vi "PIDController_AdvCalculate_FF_Sp_Pv_Per.vi"(6 "Period":dbl, 7 "Auto":bool=TRUE, 8 "FF":dbl, 9 "SP":dbl, 10 "PV":dbl, 11 "in PID_CONTROLLER":T1={"Kp"=0.0, "Ki"=0.0, "Kd"=0.0, "Period"=0.0, "Max_Integral"=0.0, "Min_Integral"=0.0, "Max_Input"=0.0, "Min_Input"=0.0, "Continuous"=FALSE, "PositionError"=0.0, "VelocityError"=0.0, "PrevError"=0.0, "Total_Integral"=0.0, "PositionTolerance"=0.0, "VelocityTolerance"=0.0, "SetPoint"=0.0, "Kf"=0.0, "Prev_Deriv"=0.0, "Prev_Deriv 2"=0.0, "DerivativeFilter"=FALSE, "Min_Output"=-9.99e+35, "Max_Output"=9.9e+35, "Prev_F_P"=0.0, "Prev_F_P_2"=0.0, "AntiWindupActive"=FALSE, "Measurement"=0.0, "IntegralZone"=9.9e+30} {"IntegralZone" format="%16_6e"; "Measurement" format="%16_6e"; "Prev_F_P_2" format="%16_6e"; "Prev_F_P" format="%16_6e"; "Max_Output" format="%16_6e"; "Min_Output" format="%16_6e"; "Prev_Deriv 2" format="%16_6e"; "Prev_Deriv" format="%16_6e"; "Kf" format="%16_6e"; "SetPoint" format="%16_6e"; "VelocityTolerance" format="%16_6e"; "PositionTolerance" format="%16_6e"; "Total_Integral" format="%16_6e"; "PrevError" format="%16_6e"; "VelocityError" format="%16_6e"; "PositionError" format="%16_6e"; "Min_Input" format="%16_6e"; "Max_Input" format="%16_6e"; "Min_Integral" format="%16_6e"; "Max_Integral" format="%16_6e"; "Period" format="%16_6e"; "Kd" format="%16_6e"; "Ki" format="%16_6e"; "Kp" format="%16_6e"}) -> (1 "ControlOutput":dbl, 3 "out PID_CONTROLLER":T1={"Kp"=0.0, "Ki"=0.0, "Kd"=0.0, "Period"=0.0, "Max_Integral"=0.0, "Min_Integral"=0.0, "Max_Input"=0.0, "Min_Input"=0.0, "Continuous"=FALSE, "PositionError"=0.0, "VelocityError"=0.0, "PrevError"=0.0, "Total_Integral"=0.0, "PositionTolerance"=0.0, "VelocityTolerance"=0.0, "SetPoint"=0.0, "Kf"=0.0, "Prev_Deriv"=0.0, "Prev_Deriv 2"=0.0, "DerivativeFilter"=FALSE, "Min_Output"=-9.99e+35, "Max_Output"=9.9e+35, "Prev_F_P"=0.0, "Prev_F_P_2"=0.0, "AntiWindupActive"=FALSE, "Measurement"=0.0, "IntegralZone"=9.9e+30} {"IntegralZone" format="%16_6e"; "Measurement" format="%16_6e"; "Prev_F_P_2" format="%16_6e"; "Prev_F_P" format="%16_6e"; "Max_Output" format="%16_6e"; "Min_Output" format="%16_6e"; "Prev_Deriv 2" format="%16_6e"; "Prev_Deriv" format="%16_6e"; "Kf" format="%16_6e"; "SetPoint" format="%16_6e"; "VelocityTolerance" format="%16_6e"; "PositionTolerance" format="%16_6e"; "Total_Integral" format="%16_6e"; "PrevError" format="%16_6e"; "VelocityError" format="%16_6e"; "PositionError" format="%16_6e"; "Min_Input" format="%16_6e"; "Max_Input" format="%16_6e"; "Min_Integral" format="%16_6e"; "Max_Integral" format="%16_6e"; "Period" format="%16_6e"; "Kd" format="%16_6e"; "Ki" format="%16_6e"; "Kp" format="%16_6e"})   [LabVIEW 2019, in "Trajectory_Library.lvlib"]
doc: "Returns the next output of the \"advanced\" PID controller. This controller implements the same PID as the \"normal\" controller with the following enhancements:\n - Integration by trapezoids is used.\n - Optionally filters derivative terms. (See SetDerivativeFilter subVI documentation for information.)\n - Incorporates optional feedforward.\n - Includes integral windup protection. This is only useful when output limits are specified.\n - When not called with a specific period, uses the actual elapsed time. (This subVI requires the call to pass the time period.) \n - Limits the outputs. When output limits are specified the output is cooerced be within these limits.\n - Includes an Auto/Manual mode. In manual mode the scaled feedforward is sent directly to the output and the PID controller tracks this output value to allow for smooth transition back to auto mode.\n\nThe generalized equation for this PID when in auto is:\n CO = Kf x feedforward + Kp x error + Ki x Integral(error) + Kd x Derivative(error)\n\nWhen auto mode is disabled, the generaized equation is:\n CO = Kf x feedforward \n \nInputs:\n - PID_Controller -- PID_Controller data cluster\n - PV-measurement -- The current measurement of the process variable. (PV)\n - SP-setpoint -- The new setpoint of the controller. (SP)\n - FF-feedforward -- Feedforward n the same units as the PV and SP\n - Period -- Period of this controller in seconds.\n - Auto -- Use the PID calculate when this is True\n\nOutputs:\n - PID_Controller -- Updated PID_Controller data cluster\n - CO-ControlOutput -- Controller output (CO)"
uses:
  Trajectory_Library.lvlib
  TypeDef/PID_CONTROLLER.ctl
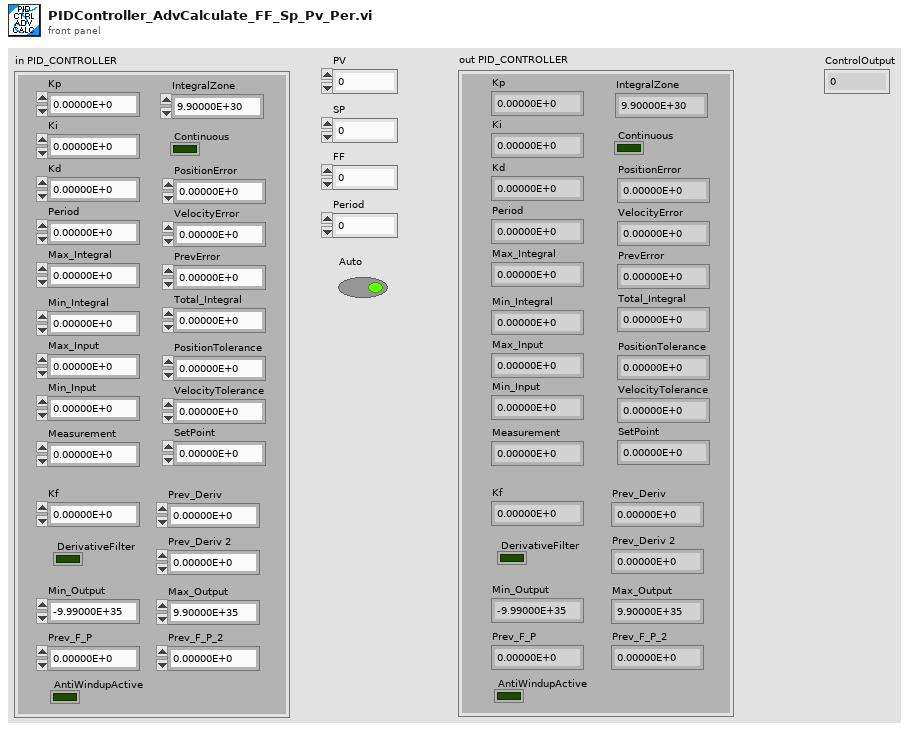
[diagram p1: front panel]
types:
  T1 = typedef "Trajectory_Library.lvlib/PID_CONTROLLER.ctl" = cluster{"Kp":dbl, "Ki":dbl, "Kd":dbl, "Period":dbl, "Max_Integral":dbl, "Min_Integral":dbl, "Max_Input":dbl, "Min_Input":dbl, "Continuous":bool, "PositionError":dbl, "VelocityError":dbl, "PrevError":dbl, "Total_Integral":dbl, "PositionTolerance":dbl, "VelocityTolerance":dbl, "SetPoint":dbl, "Kf":dbl, "Prev_Deriv":dbl, "Prev_Deriv 2":dbl, "DerivativeFilter":bool, "Min_Output":dbl, "Max_Output":dbl, "Prev_F_P":dbl, "Prev_F_P_2":dbl, "AntiWindupActive":bool, "Measurement":dbl, "IntegralZone":dbl}
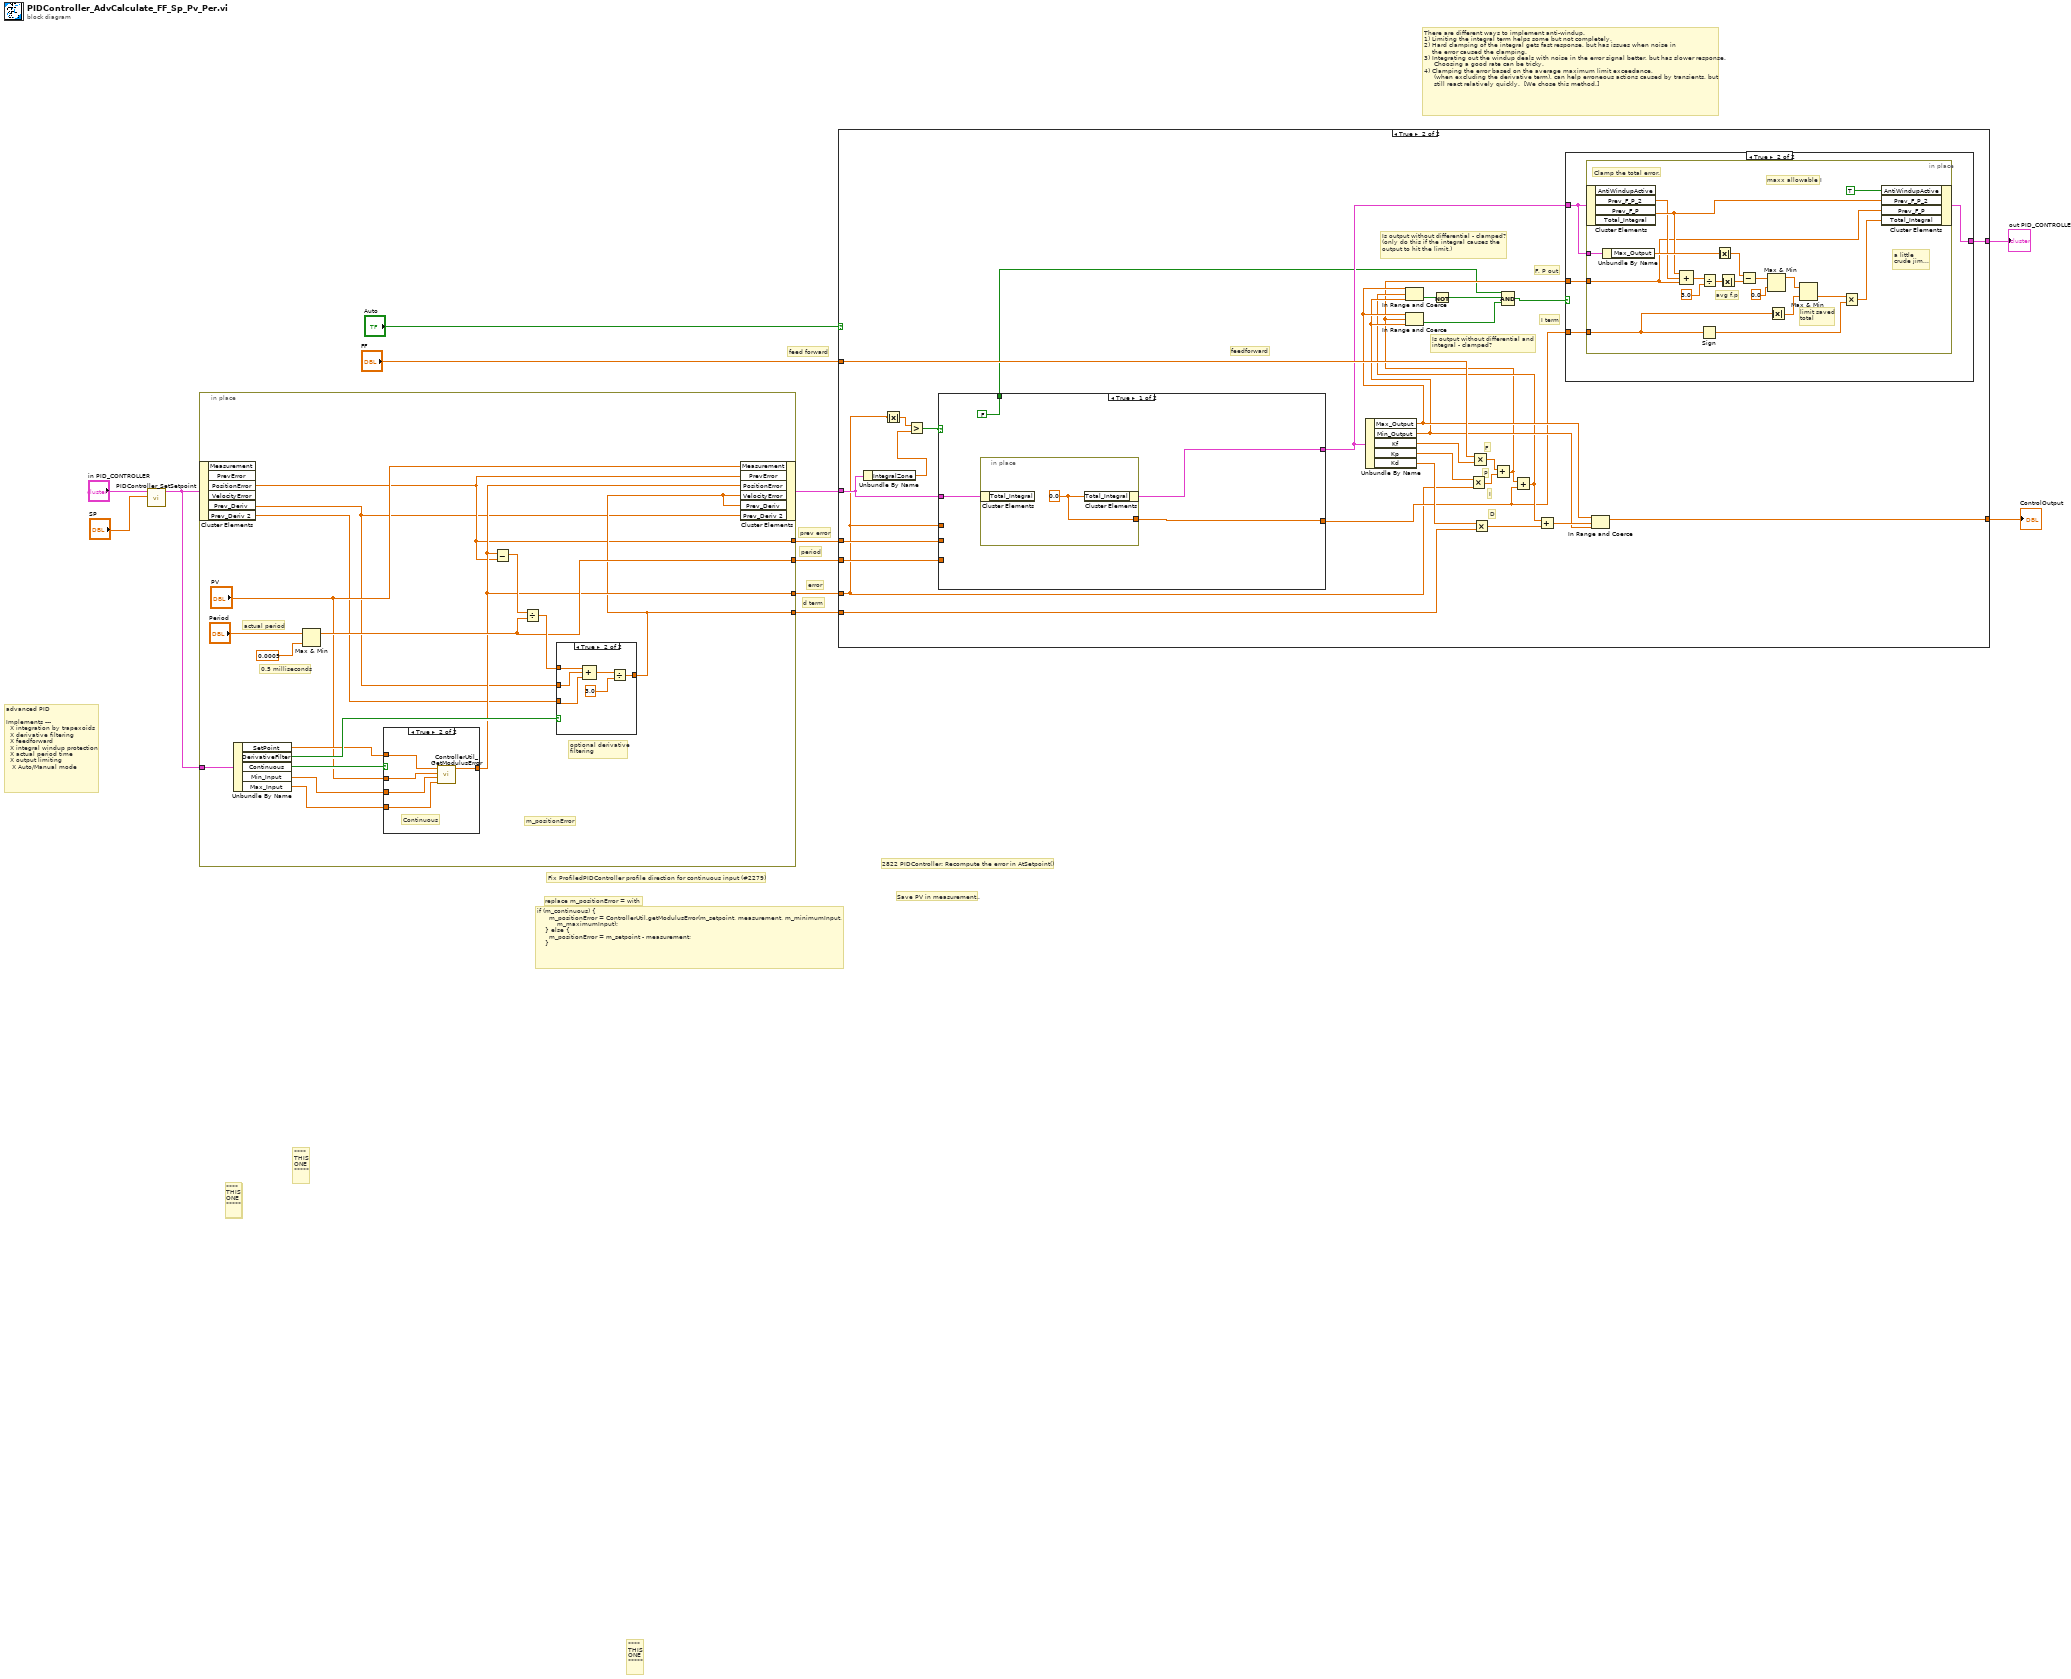
[diagram p0: block diagram]
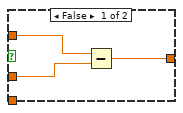
[diagram p2: hidden frame]
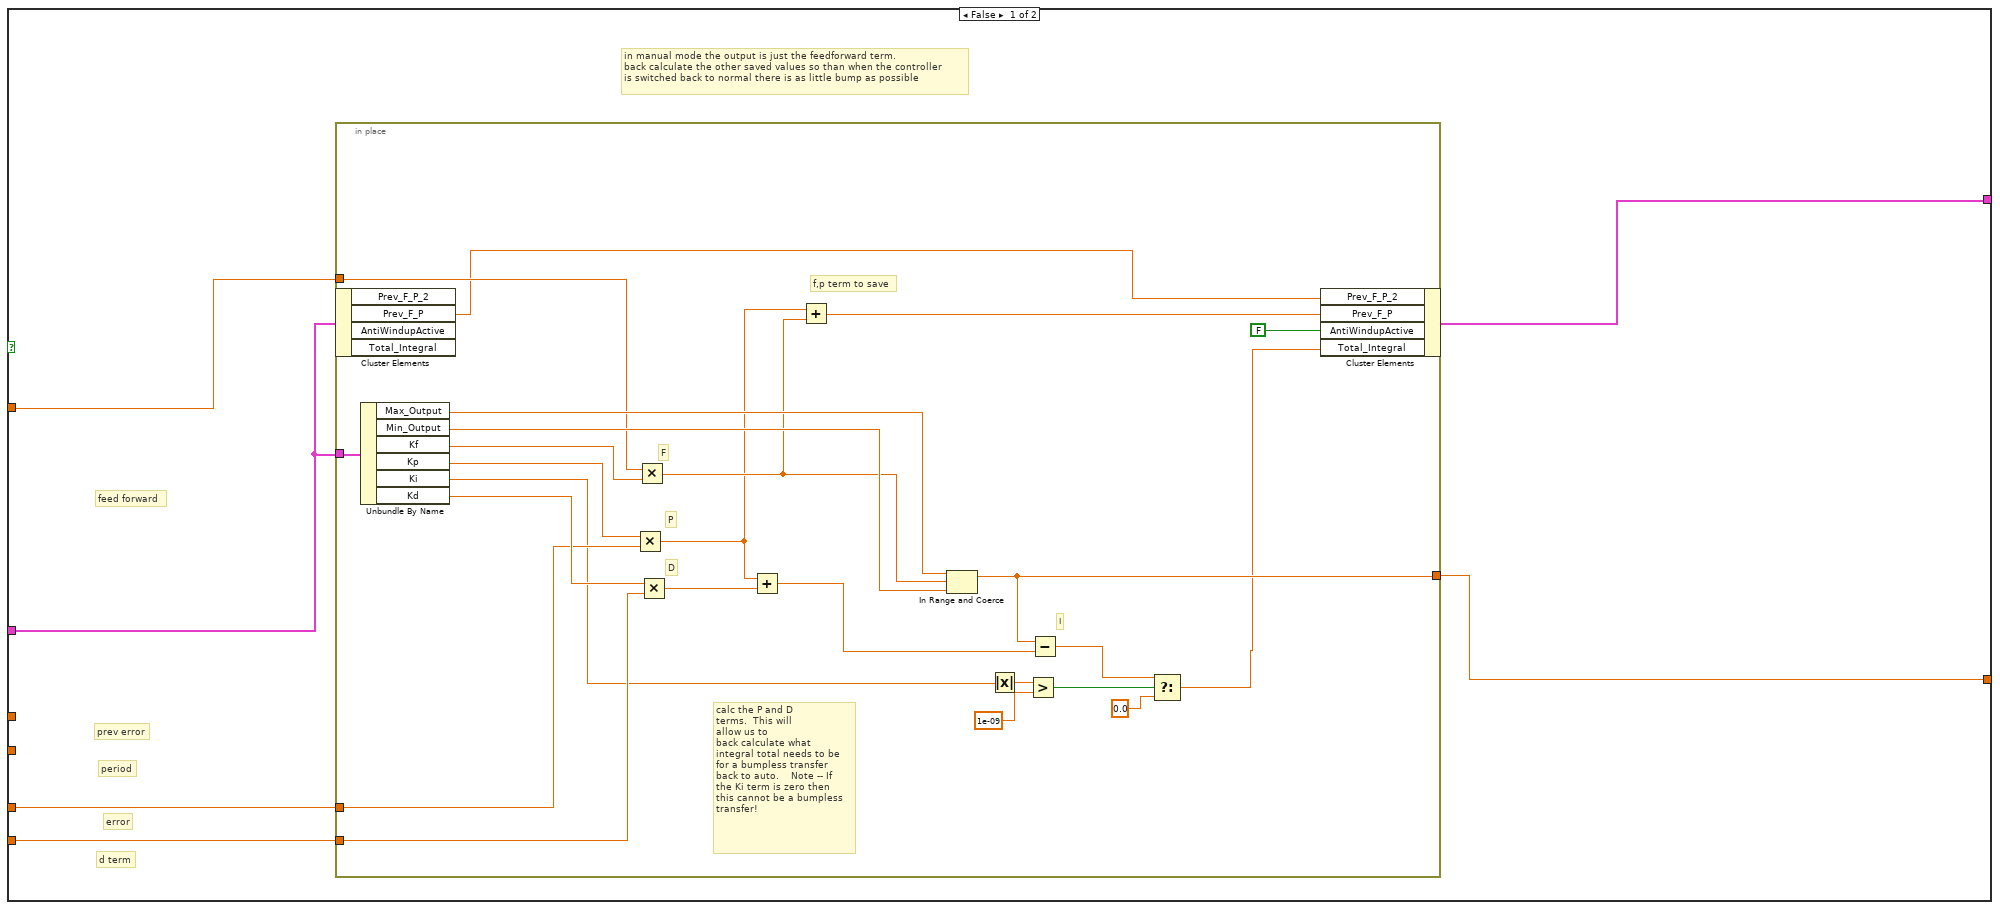
[diagram p4: hidden frame]
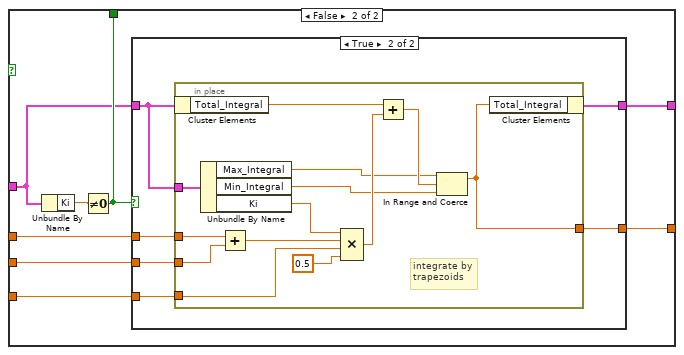
[diagram p5: hidden frame]
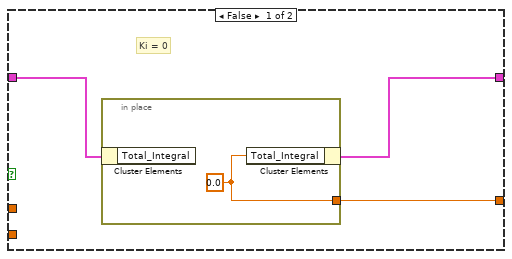
[diagram p6: hidden frame]
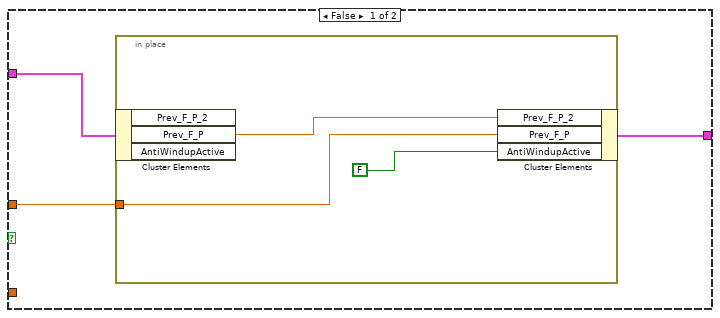
[diagram p7: hidden frame]
diagram:
  # "feed forward"
  # "prev error"
  # "period"
  # "error"
  # "d term"
  # "Save PV in measurement.."
  # "2822 PIDController: Recompute the error in AtSetpoint()"
  # "Fix ProfiledPIDController profile direction for continuous input (#2279)"
  # "replace m_positionError = with"
  # "if (m_continuous) {\n      m_positionError = ControllerUtil.getModulusError(m_setpoint, measurement, m_minimumInput,\n          m_maximumInput);\n    } else {\n      m_positionError = m_setpoint - measurement;\n    }"
  # "There are different ways to implement anti-windup. \n1) Limiting the integral term helps some but not completely.\n2) Hard clamping of the integral gets fast response, but has issues when noise in\n    the error caused the clamping.\n3) Integrating out the windup deals with noise in the error signal better, but has slower response.\n     Choosing a good rate can be tricky.\n4) Clamping the error based on the average maximum limit exceedance, \n     (when excluding the derivative term), can help erroneous actions caused by transients, but\n     still react relatively quickly.  [We chose this method.]"
  # "advanced PID\n\nImplements ---\n  X integration by trapexoids\n  X derivative filtering\n  X feedforward\n  X integral windup protection\n  X actual period time\n  X output limiting\n   X Auto/Manual mode"
  # "****\nTHIS\nONE\n*****"
  # "****\nTHIS\nONE\n*****"
  # "****\nTHIS\nONE\n*****"
  # "****\nTHIS\nONE\n*****"
  n1 = call "PIDController_SetSetpoint.vi"("Setpoint"="SP", "in PID_CONTROLLER"="in PID_CONTROLLER") -> ("out PID_CONTROLLER"=w1:T1)  [unwired: 9 in]
  n2 = in-place {
    in-place-border: [w17] -> w9
    in-place-border: [w25] -> w8
    in-place-border: [w16] -> w4
    in-place-border: [w18] -> w3
    in-place-border: w1 -> [w14]
    # "m_positionError"
    # "0.5 milliseconds"
    # "actual period"
    # "optional derivative\nfiltering"
    n3 = in-place-cluster #1(w1) -> ("PositionError"=w16:dbl, "Prev_Deriv"=w13:dbl, "Prev_Deriv 2"=w15:dbl)  [unwired: 3 out]
    n4 = Unbundle By Name(w14) -> ("SetPoint"=w23:dbl, "DerivativeFilter"=w28:bool, "Continuous"=w22:bool, "Min_Input"=w21:dbl, "Max_Input"=w20:dbl)
    n5 = Max & Min(x="Period", y=0.0005) -> (max(x,y)=w25:dbl)  [unwired: 1 out]
    n6 = case shown="True" w22 {
      tunnel: w23 -> [w32 w37]
      tunnel: "PV" -> [w31 w36]
      tunnel: [w30 w33] -> w18
      tunnel: w21 -> [_ w35]
      tunnel: w20 -> [_ w34]
      frame False {
        n7 = Subtract(x=w32, y=w31) -> (x-y=w30:dbl)
      }
      frame True {
        # "Continuous"
        n8 = call "ControllerUtil_GetModulusError.vi"("Maximum_Input"=w34, "Minimum_Input"=w35, "Measurerment(PV)"=w36, "Reference(SP)"=w37) -> ("Error"=w33:dbl)  [unwired: 7 in]
      }
    }
    n9 = Subtract(x=w18, y=w16) -> (x-y=w29:dbl)
    n10 = Divide(x=w29, y=w25) -> (x/y=w27:dbl)
    n11 = case shown="True" w28 {
      tunnel: w27 -> [w38 w44]
      tunnel: [w38 w41] -> w17
      tunnel: w15 -> [_ w43]
      tunnel: w13 -> [_ w42]
      frame False {
      }
      frame True {
        n12 = Compound Arithmetic op=ADD(w44, w42, w43) -> (w39:dbl)
        n13 = Divide(x=w39, y=3.0) -> (x/y=w41:dbl)
      }
    }
    n14 = in-place-cluster #1("Measurement"="PV", "PrevError"=w16, "PositionError"=w18, "VelocityError"=w17, "Prev_Deriv"=w17, "Prev_Deriv 2"=w13) -> (w2:T1)
  }
  n15 = case shown="True" "Auto" {
    tunnel: w4 -> [_ w101]
    tunnel: "FF" -> [w50 w100]
    tunnel: w9 -> [w49 w98]
    tunnel: w8 -> [_ w97]
    tunnel: [w47 w96] -> w7
    tunnel: [w45 w94] -> w6
    tunnel: w2 -> [w46 w77]
    tunnel: w3 -> [w48 w75]
    frame False {
      # "in manual mode the output is just the feedforward term.\nback calculate the other saved values so than when the controller\nis switched back to normal there is as little bump as possible"
      # "prev error"
      # "period"
      # "error"
      # "d term"
      # "feed forward"
      n16 = in-place {
        in-place-border: w50 -> [w68]
        in-place-border: w49 -> [w67]
        in-place-border: w48 -> [w66]
        in-place-border: [w65] -> w47
        in-place-border: w46 -> [w61]
        # "f,p term to save"
        # "I"
        # "calc the P and D\nterms.  This will \nallow us to \nback calculate what\nintegral total needs to be\nfor a bumpless transfer\nback to auto.    Note -- If\nthe Ki term is zero then \nthis cannot be a bumpless\ntransfer!"
        # "D"
        # "P"
        # "F"
        n17 = in-place-cluster #2(w46) -> ("Prev_F_P"=w55:dbl)  [unwired: 3 out]
        n18 = Unbundle By Name(w61) -> ("Max_Output"=w70:dbl, "Min_Output"=w69:dbl, "Kf"=w72:dbl, "Kp"=w74:dbl, "Ki"=w58:dbl, "Kd"=w73:dbl)
        n19 = Multiply(x=w74, y=w66) -> (x*y=w62:dbl)
        n20 = Multiply(x=w68, y=w72) -> (x*y=w63:dbl)
        n21 = Multiply(x=w73, y=w67) -> (x*y=w71:dbl)
        n22 = Add(x=w62, y=w71) -> (x+y=w64:dbl)
        n23 = Add(x=w62, y=w63) -> (x+y=w57:dbl)
        n24 = In Range and Coerce(upper limit=w70, x=w63, lower limit=w69) -> (coerced(x)=w65:dbl)  [unwired: 1 out]
        n25 = Absolute Value(x=w58) -> (abs(x)=w60:dbl)
        n26 = Greater?(x=w60, y=1e-09) -> (0:w54:bool)
        n27 = Subtract(x=w65, y=w64) -> (x-y=w53:dbl)
        n28 = Select(t=w53, s=w54, f=0.0) -> (s? t:f=w52:dbl)
        n29 = in-place-cluster #2("Prev_F_P_2"=w55, "Prev_F_P"=w57, "AntiWindupActive"=FALSE, "Total_Integral"=w52) -> (w45:T1)
      }
    }
    frame True {
      # "I term"
      # "F, P out"
      # "D"
      # "I"
      # "P"
      # "F"
      # "Is output without differential and \nintegral - clamped?"
      # "Is output without differential - clamped?\n(only do this if the integral causes the \noutput to hit the limit.)"
      # "feedforward"
      n30 = Unbundle By Name(w77) -> ("IntegralZone"=w76:dbl)
      n31 = Absolute Value(x=w75) -> (abs(x)=w80:dbl)
      n32 = Greater?(x=w80, y=w76) -> (0:w79:bool)
      n33 = case shown="True" w79 {
        tunnel: [w105 w115] -> w78
        tunnel: w101 -> [_ w114]
        tunnel: w97 -> [_ w113]
        tunnel: [w106 w112] -> w95
        tunnel: [FALSE w111] -> w81
        tunnel: w77 -> [w107 w110]
        tunnel: w75 -> [_ w109]
        frame True {
          n34 = in-place {
            in-place-border: [w108] -> w105
            w108 = 0.0 ("TotalError")
            n35 = in-place-cluster #3(w107) -> ()  [unwired: 1 out]
            n36 = in-place-cluster #3("Total_Integral"=w108) -> (w106:T1)
          }
        }
        frame False {
          n37 = Unbundle By Name(w110) -> ("Ki"=w116:dbl)
          n38 = Not Equal To 0?(x=w116) -> (x != 0?=w111:bool)
          n39 = case shown="True" w111 {
            tunnel: w110 -> [w118 w122]
            tunnel: [w117 w121] -> w112
            tunnel: [w119 w126] -> w115
            tunnel: w113 -> [_ w123]
            tunnel: w109 -> [_ w125]
            tunnel: w114 -> [_ w124]
            frame False {
              # "Ki = 0"
              n40 = in-place {
                in-place-border: [w120] -> w119
                w120 = 0.0 ("Total_Integral")
                n41 = in-place-cluster #4(w118) -> ()  [unwired: 1 out]
                n42 = in-place-cluster #4("Total_Integral"=w120) -> (w117:T1)
              }
            }
            frame True {
              n43 = in-place {
                in-place-border: w122 -> [w138]
                in-place-border: [w128] -> w126
                in-place-border: w125 -> [w137]
                in-place-border: w124 -> [w136]
                in-place-border: w123 -> [w134]
                # "integrate by\ntrapezoids"
                n44 = in-place-cluster #5(w122) -> ("Total_Integral"=w127:dbl)
                n45 = Unbundle By Name(w138) -> ("Max_Integral"=w131:dbl, "Min_Integral"=w130:dbl, "Ki"=w129:dbl)
                n46 = Add(x=w137, y=w136) -> (x+y=w135:dbl)
                n47 = Compound Arithmetic op=MULTIPLY(w129, w135, w134, 0.5 ("value")) -> (w132:dbl)
                n48 = Add(x=w127, y=w132) -> (x+y=w139:dbl)
                n49 = In Range and Coerce(upper limit=w131, x=w139, lower limit=w130) -> (coerced(x)=w128:dbl)  [unwired: 1 out]
                n50 = in-place-cluster #5("Total_Integral"=w128) -> (w121:T1)
              }
            }
          }
        }
      }
      n51 = Unbundle By Name(w95) -> ("Max_Output"=w89:dbl, "Min_Output"=w88:dbl, "Kf"=w99:dbl, "Kp"=w103:dbl, "Kd"=w102:dbl)
      n52 = Multiply(x=w103, y=w75) -> (x*y=w90:dbl)
      n53 = Multiply(x=w100, y=w99) -> (x*y=w91:dbl)
      n54 = Multiply(x=w102, y=w98) -> (x*y=w92:dbl)
      n55 = Add(x=w91, y=w90) -> (x+y=w82:dbl)
      n56 = In Range and Coerce(upper limit=w89, x=w82, lower limit=w88) -> (In Range?=w85:bool)  [unwired: 1 out]
      n57 = Add(x=w82, y=w78) -> (x+y=w83:dbl)
      n58 = In Range and Coerce(upper limit=w89, x=w83, lower limit=w88) -> (In Range?=w87:bool)  [unwired: 1 out]
      n59 = Not(x=w87) -> (.not. x?=w86:bool)
      n60 = Compound Arithmetic op=AND(w81, w86, w85) -> (w84:bool)
      n61 = Add(x=w83, y=w92) -> (x+y=w93:dbl)
      n62 = case shown="True" w84 {
        tunnel: w95 -> [w141 w147]
        tunnel: [w140 w146] -> w94
        tunnel: w78 -> [_ w148]
        tunnel: w82 -> [w142 w149]
        frame False {
          n63 = in-place {
            in-place-border: w142 -> [w143]
            n64 = in-place-cluster #6(w141) -> ("Prev_F_P"=w145:dbl)  [unwired: 2 out]
            n65 = in-place-cluster #6("Prev_F_P_2"=w145, "Prev_F_P"=w143, "AntiWindupActive"=FALSE) -> (w140:T1)
          }
        }
        frame True {
          n66 = in-place {
            in-place-border: w147 -> [w168]
            in-place-border: w149 -> [w151]
            in-place-border: w148 -> [w158]
            # "limit saved\ntotal"
            # "maxx allowable I"
            # "a little\ncrude jim..."
            # "avg f,p"
            # "Clamp the total error."
            n67 = in-place-cluster #7(w147) -> ("Prev_F_P_2"=w152:dbl, "Prev_F_P"=w153:dbl)  [unwired: 2 out]
            n68 = Unbundle By Name(w168) -> ("Max_Output"=w164:dbl)
            n69 = Compound Arithmetic op=ADD(w153, w152, w151) -> (w167:dbl)
            n70 = Sign(1:w158) -> (0:w161:dbl)
            n71 = Divide(x=w167, y=3.0) -> (x/y=w165:dbl)
            n72 = Absolute Value(x=w164) -> (abs(x)=w159:dbl)
            n73 = Absolute Value(x=w165) -> (abs(x)=w160:dbl)
            n74 = Subtract(x=w159, y=w160) -> (x-y=w163:dbl)
            n75 = Max & Min(x=w163, y=0.0) -> (max(x,y)=w157:dbl)  [unwired: 1 out]
            n76 = Absolute Value(x=w158) -> (abs(x)=w156:dbl)
            n77 = Max & Min(x=w157, y=w156) -> (min(x,y)=w155:dbl)  [unwired: 1 out]
            n78 = Multiply(x=w155, y=w161) -> (x*y=w150:dbl)
            n79 = in-place-cluster #7("AntiWindupActive"=TRUE, "Prev_F_P_2"=w153, "Prev_F_P"=w151, "Total_Integral"=w150) -> (w146:T1)
          }
        }
      }
      n80 = In Range and Coerce(upper limit=w89, x=w93, lower limit=w88) -> (coerced(x)=w96:dbl)  [unwired: 1 out]
    }
  }
  "out PID_CONTROLLER" <- w6
  "ControlOutput" <- w7
